vi "Get XML.vi"(8 "error in (no error)":errorcluster, 11 "reference":refnum<k24>) -> (0 "error out":errorcluster, 2 "GetContent":string, 3 "reference out":refnum<k24>)   [LabVIEW 2026, in "ToastNotification.lvlib" / "Toast Native.lvlib"]
doc: "Serialize a borrowed native ToastContent as XML. GetContent is a copied LabVIEW string. reference out aliases the input content handle and must not be closed separately as a second acquisition. The owner of the content handle closes it after serialization."
uses:
  Toast Native.lvlib
  C:/Users/loicw/Documents/LabVIEW/ToastNotifications/Sources/bins/Microsoft.Toolkit.Uwp.Notifications.dll
  bins/Microsoft.Toolkit.Uwp.Notifications.dll
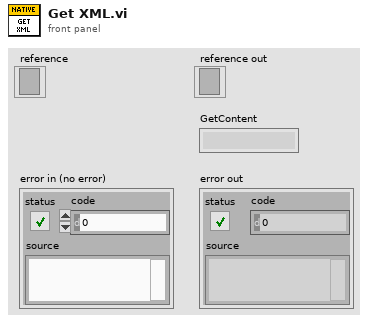
[diagram p1: front panel]
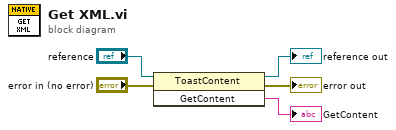
[diagram p0: block diagram]
diagram:
  n1 = invoke class="ToastContent" method="GetContent"(reference="reference", error in="error in (no error)") -> (reference out=→"reference out":refnum<k24>, error out=→"error out":errorcluster, "GetContent"=→"GetContent":string)  [unwired: 1 in]
